vi "LoadQ0File.vi"(8 "error in (no error)":errorcluster, 10 "Q0 external file":path, 11 "Scope5761 in":refnum<class "Scope5782_six_channel.lvclass">) -> (0 "error out":errorcluster, 3 "Scope5761 out":refnum<class "Scope5782_six_channel.lvclass">)   [LabVIEW 2025, in "Scope5782_six_channel.lvclass"]
uses:
  Scope5782_six_channel.lvclass
  Scope5782_six_channel.lvclass/Scope5782_six_channel.ctl
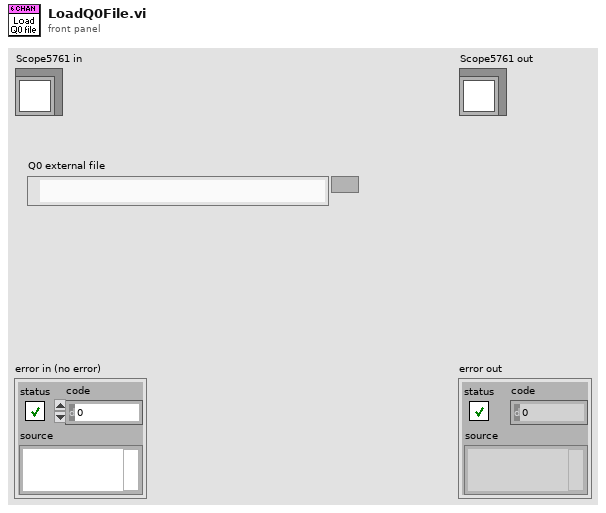
[diagram p1: front panel]
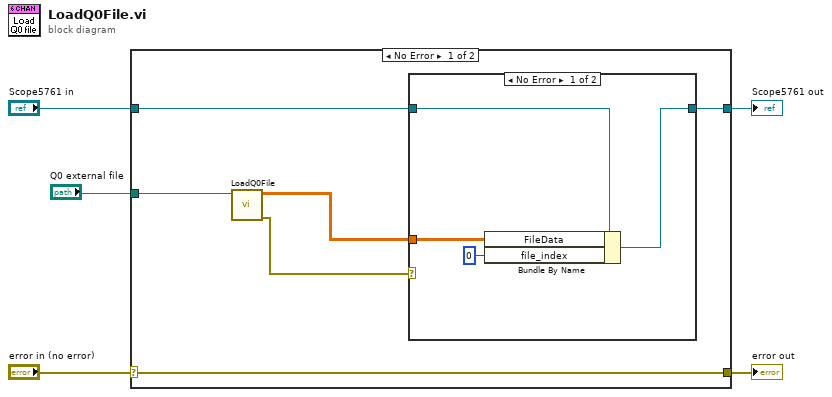
[diagram p0: block diagram]
diagram:
  n1 = case shown="No Error" "error in (no error)" {
    selector: "error in (no error)" -> [w11 w18]
    tunnel: [w11 w18] -> w4
    tunnel: [w7 w17] -> w2
    tunnel: "Scope5761 in" -> [w8 w17]
    tunnel: "Q0 external file" -> [w10 _]
    frame No Error {
      n2 = call "LoadQ0File.vi"("Q0 external file"=w10) -> ("error out"=w6:errorcluster, "FileData"=w9:dbl[][])  [unwired: 9 in]
      n3 = case shown="No Error" w6 {
        tunnel: w9 -> [w14 _]
        tunnel: w8 -> [w13 w16]
        tunnel: [w12 w16] -> w7
        frame No Error {
          n4 = Bundle By Name(cluster=w13, "FileData"=w14, "file_index"=0 ("Q0 registers.file_index")) -> (w12:refnum<class "Scope5782_six_channel.lvclass">)
        }
        frame Error {
        }
      }
    }
    frame Error {
    }
  }
  "error out" <- w4
  "Scope5761 out" <- w2
